vi "Initialize.vi"(8 "error in (no error)":errorcluster caption="错误输入（无错误）", 9 "Module ID":i32, 10 "Reference":T1, 11 "Data Viewer 输入":refnum<class "Data Viewer.lvclass">) -> (0 "error out":errorcluster caption="错误输出", 3 "Data Viewer 输出":refnum<class "Data Viewer.lvclass">)   [LabVIEW 2020, in "Data Viewer.lvlib" / "Data Viewer.lvclass"]
uses:
  Data Viewer.lvclass
  Control Reference.ctl
  Legend.ctl
  Filter Arguments.ctl
  Filter Type.ctl
  Filter Method.ctl
  Data Viewer.lvclass/Data Viewer.ctl
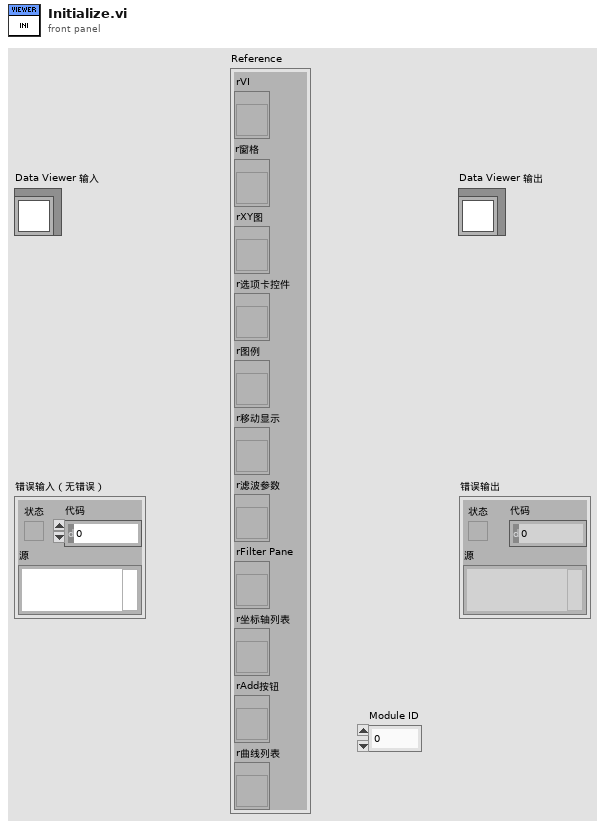
[diagram p1: front panel]
types:
  T1 = typedef "Data Viewer.lvlib/Data Viewer.lvclass/Control Reference.ctl" = cluster{"rVI":refnum<vi>, "r窗格":refnum<vi>, "rXY图":refnum<vi>, "r选项卡控件":refnum<vi>, "r图例":refnum<vi>, "r移动显示":refnum<vi>, "r滤波参数":refnum<vi>, "rFilter Pane ":refnum<vi>, "r坐标轴列表":refnum<vi>, "rAdd按钮":refnum<vi>, "r曲线列表":refnum<vi>}
  T2 = typedef "Data Viewer.lvlib/Data Viewer.lvclass/Filter Type.ctl" = enum16{"Butterworth滤波器", "中值滤波器"}
  T3 = typedef "Data Viewer.lvlib/Data Viewer.lvclass/Legend.ctl" = cluster{"颜色":u32, "曲线名称":string}[]
  T4 = cluster{"Curve":i32, "Point":cluster{"X":dbl, "Y":dbl}}
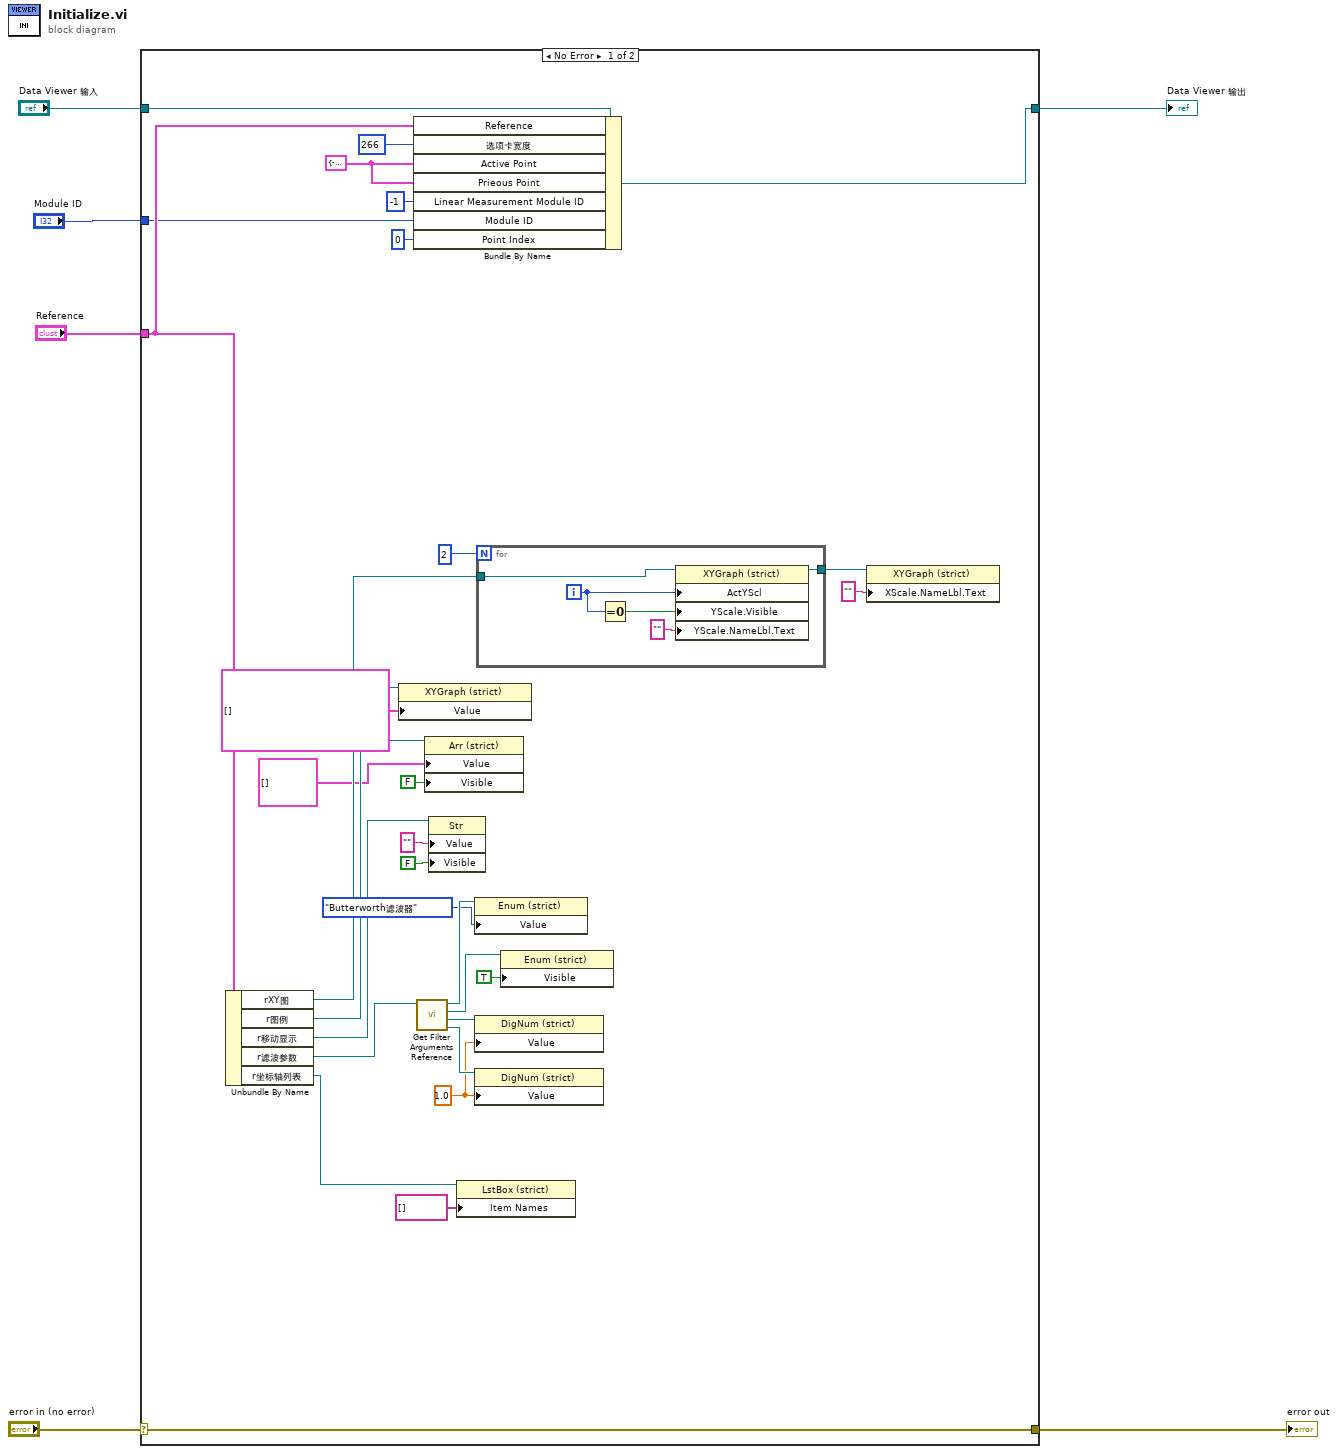
[diagram p0: block diagram]
diagram:
  n1 = case shown="No Error" "error in (no error)" {
    selector: "error in (no error)" -> [w35 w43]
    tunnel: [w35 w43] -> w5
    tunnel: [w34 w42] -> w3
    tunnel: "Data Viewer 输入" -> [w36 w42]
    tunnel: "Reference" -> [w32 _]
    tunnel: "Module ID" -> [w11 _]
    frame No Error {
      w13 = T4 {"Curve"=-1, "Point"={"X"=0.0, "Y"=0.0}} ("Active Point")
      w16 = 1.0 ("值")
      n2 = Unbundle By Name(w32) -> ("rXY图"=w30:refnum<vi>, "r图例"=w27:refnum<vi>, "r移动显示"=w24:refnum<vi>, "r滤波参数"=w21:refnum<vi>, "r坐标轴列表"=w9:refnum<vi>)
      n3 = property class="XYGraph (strict)"(reference=w30, "Value"=cluster{"Time":timestamp[], "Value":dbl[]}[] []) -> ()  [unwired: 1 in, 2 out]
      n4 = Bundle By Name(cluster=w36, "Reference"=w32, "选项卡宽度"=u32 266, "Active Point"=w13, "Prieous Point"=w13, "Linear Measurement Module ID"=-1, "Module ID"=w11, "Point Index"=0) -> (w34:refnum<class "Data Viewer.lvclass">)
      n5 = call "Get Filter Arguments Reference.vi"("滤波参数引用"=w21) -> ("参数2"=w17:refnum<vi>, "参数1"=w18:refnum<vi>, "滤波方式"=w19:refnum<vi>, "滤波器类型"=w20:refnum<vi>)  [unwired: 7 in]
      n6 = property class="Arr (strict)"(reference=w27, "Value"=T3 [] ("值"), "Visible"=FALSE ("可见")) -> ()  [unwired: 1 in, 2 out]
      n7 = property class="Str"(reference=w24, "Value"="" ("值"), "Visible"=FALSE ("可见")) -> ()  [unwired: 1 in, 2 out]
      n8 = property class="LstBox (strict)"(reference=w9, "Item Names"=string[] []) -> ()  [unwired: 1 in, 2 out]
      n9 = property class="Enum (strict)"(reference=w20, "Value"=Filter_Type."Butterworth滤波器" ("值")) -> ()  [unwired: 1 in, 2 out]
      n10 = property class="DigNum (strict)"(reference=w18, "Value"=w16) -> ()  [unwired: 1 in, 2 out]
      n11 = property class="DigNum (strict)"(reference=w17, "Value"=w16) -> ()  [unwired: 1 in, 2 out]
      n12 = for {
        N: 2 -> [_]
        tunnel: w30 -> [w41]
        tunnel: [w37] -> w29
        i -> [w40]
        n13 = Equal To 0?(x=w40) -> (x = 0?=w39:bool)
        n14 = property class="XYGraph (strict)"(reference=w41, "ActYScl"=w40, "YScale.Visible"=w39, "YScale.NameLbl.Text"="" ("Y标尺.名称标签.文本")) -> (reference out=w37:refnum<vi>)  [unwired: 1 in, 1 out]
      }
      n15 = property class="Enum (strict)"(reference=w19, "Visible"=TRUE ("可见")) -> ()  [unwired: 1 in, 2 out]
      n16 = property class="XYGraph (strict)"(reference=w29, "XScale.NameLbl.Text"="" ("X标尺.名称标签.文本")) -> ()  [unwired: 1 in, 2 out]
    }
    frame Error {
    }
  }
  "error out" <- w5
  "Data Viewer 输出" <- w3
